vi "Logger Stopped.vi"(8 "error in (no error)":errorcluster, 10 "Logger Stopped":T1, 11 "Log Manager Module in":refnum<class "Log Manager Module.lvclass">) -> (0 "error out":errorcluster, 3 "Log Manager Module out":refnum<class "Log Manager Module.lvclass">)   [LabVIEW 2020, in "VolatusData.lvlib" / "Log Manager Module.lvclass"]
uses:
  Log Manager Module.lvclass
  Log Manager Module.lvclass/Log Manager Module.ctl
  Logger State.ctl
  VolatusData.lvlib
  Volatus/Module/Module.lvclass
  Volatus/Event Level.ctl
  Volatus/Volatus.lvlib
  C:/dev/lv20CE/gpack-tests/lv-volatus/Volatus/Module/Module.lvclass
  C:/dev/lv20CE/gpack-tests/lv-volatus/VolatusData/Log Manager Module/Log Manager Module.lvclass
  Logger Stopped.ctl
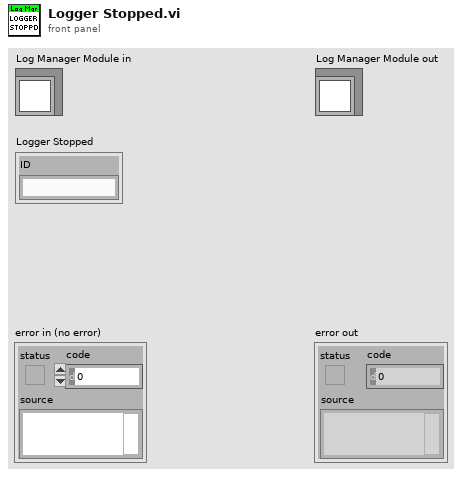
[diagram p1: front panel]
types:
  T1 = typedef "VolatusData.lvlib/Logger Stopped.ctl" = cluster{"ID":string}
  T2 = typedef "VolatusData.lvlib/Logger State.ctl" = enum16{"Unknown", "Idle", "Preparing", "Ready", "Logging", "Stopping"}
  T3 = typedef "VolatusData.lvlib/Log Manager Module.lvclass/Group Info.ctl" = cluster{"Name":string, "Loggers":map{string, T4}}
  T4 = typedef "VolatusData.lvlib/Log Manager Module.lvclass/Logger.ctl" = cluster{"ID":string, "MsgQ":refnum<class "MessageQ.lvclass">, "State":T2, "Group":string}
  T5 = typedef "Volatus.lvlib/Event Level.ctl" = enum16{"Debug", "Info", "Warning", "Error"}
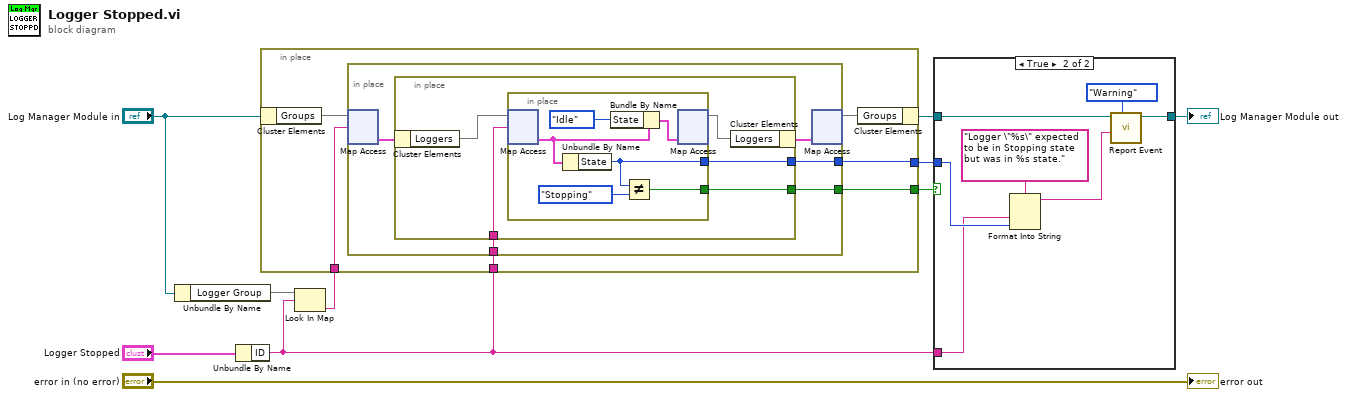
[diagram p0: block diagram]
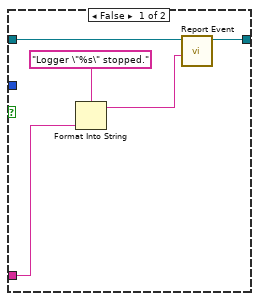
[diagram p2: hidden frame]
diagram:
  n1 = Unbundle By Name("Log Manager Module in") -> ("Logger Group"=w3:map{string, string})
  n2 = Unbundle By Name("Logger Stopped") -> ("ID"=w2:string)
  n3 = Look In Map(map=w3, key=w2) -> (value=w1:string)  [unwired: 1 in, 1 out]
  n4 = in-place {
    in-place-border: w2 -> [w16]
    in-place-border: [w15] -> w6
    in-place-border: [w14] -> w5
    in-place-border: w1 -> [w12]
    n5 = in-place-cluster #1("Log Manager Module in") -> ("Groups"=w13:map{string, T3})
    n6 = in-place {
      in-place-border: w16 -> [w21]
      in-place-border: [w20] -> w15
      in-place-border: [w19] -> w14
      n7 = in-place-map #2(w13, w12) -> (w18:T3)  [unwired: 1 in, 1 out]
      n8 = in-place {
        in-place-border: w21 -> [w26]
        in-place-border: [w25] -> w20
        in-place-border: [w24] -> w19
        n9 = in-place-cluster #3(w18) -> ("Loggers"=w23:map{string, T4})
        n10 = in-place {
          in-place-border: [w28] -> w25
          in-place-border: [w27] -> w24
          n11 = in-place-map #4(w23, w26) -> (w30:T4)  [unwired: 1 in, 1 out]
          n12 = Unbundle By Name(w30) -> ("State"=w27:T2)
          n13 = Bundle By Name(cluster=w30, "State"=Logger_State."Idle") -> (w31:T4)
          n14 = Not Equal?(x=w27, y=Logger_State."Stopping") -> (x != y?=w28:bool)
          n15 = in-place-map #4(w31) -> (w22:map{string, T4})  [unwired: 1 in, 2 out]
        }
        n16 = in-place-cluster #3("Loggers"=w22) -> (w17:T3)
      }
      n17 = in-place-map #2(w17) -> (w11:map{string, T3})  [unwired: 1 in, 2 out]
    }
    n18 = in-place-cluster #1("Groups"=w11) -> (w8:refnum<class "Log Manager Module.lvclass">)
  }
  n19 = case shown="True" w6 {
    tunnel: w8 -> [w37 w44]
    tunnel: [w36 w42] -> w7
    tunnel: w5 -> [_ w40]
    tunnel: w2 -> [w34 w39]
    frame False {
      n20 = Format Into String(format string="Logger \"%s\" stopped.", w34) -> (resulting string=w33:string)  [unwired: 2 in, 1 out]
      n21 = call "Report Event.vi"("Message"=w33, "Module in"=w37) -> ("Module out"=w36:refnum<class "Log Manager Module.lvclass">)  [unwired: 8 in, 1 out]
    }
    frame True {
      n22 = Format Into String(format string="Logger \"%s\" expected to be in Stopping state but was in %s state.", w39, w40) -> (resulting string=w38:string)  [unwired: 2 in, 1 out]
      n23 = call "Report Event.vi"("Level (Info)"=Event_Level."Warning", "Message"=w38, "Module in"=w44) -> ("Module out"=w42:refnum<class "Log Manager Module.lvclass">)  [unwired: 7 in, 1 out]
    }
  }
  "Log Manager Module out" <- w7
  "error out" <- "error in (no error)"
